vi "Two Way Event Recorder Init VISA Comms.vi"(8 "error in (no error)":errorcluster, 11 "Device Ref in":T1 format="%.0x") -> (0 "error out":errorcluster, 3 "Visa reference out":refnum<visa-resource-name>)   [LabVIEW 2017, in "Two Way Event Recorder Custom Device.lvlib"]
uses:
  Two Way Event Recorder Custom Device.lvlib
  <vilib>/NI Veristand/Custom Device API/Custom Device Item Ref.ctl
  Two Way Event Recorder Property Lookup.vi
  <vilib>/NI Veristand/Custom Device API/Get Item Property (String).vi
  <vilib>/NI Veristand/Custom Device API/Get Item Property (U32).vi
  <vilib>/NI Veristand/Custom Device API/Get Item Property (U16).vi
  <vilib>/NI Veristand/Custom Device API/Custom Device API.lvlib
panel:
  in  "Serial Settings:Wire Mode":i16(ring)=-1 items=["Unknown"=-1, "RS485/Wire4"=0, "RS485/Wire2-EchoDTR"=1, "RS485/Wire2-CtrlDTR"=2, "RS485/Wire2-Auto"=3, "RS232/DTE"=128, "RS232/DCE"=129, "RS232/Auto"=130]
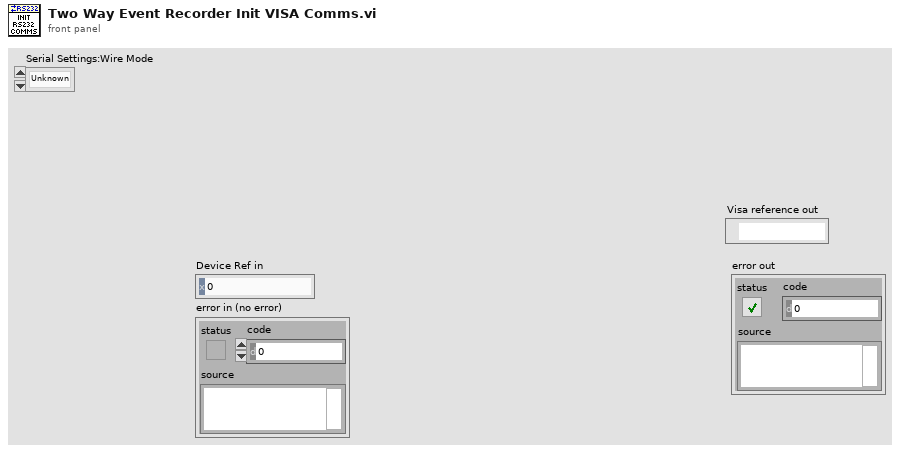
[diagram p1: front panel]
types:
  T1 = typedef "Custom Device API.lvlib/Custom Device Item Ref.ctl" = u64
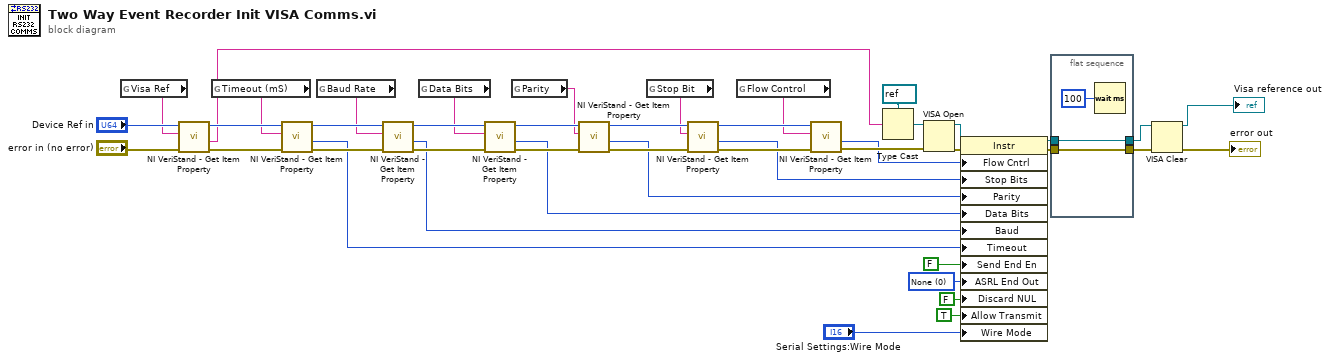
[diagram p0: block diagram]
diagram:
  w4 = u16 0 items=["None", "Last Bit", "TermChar", "Break"] ("Serial Settings:End Mode for Writes")
  n1 = global read "Two Way Event Recorder Property Lookup.vi" "Visa Ref"() -> (w18:string)
  n2 = call-poly <vilib>:"NI VeriStand - Get Item Property.vi"("error in (no error)"="error in (no error)", "Property Name"=w18, "Item Ref in"="Device Ref in") -> ("error out"=w42:errorcluster, "Value"=w31:string, "Item Ref out"=w44:T1)  [unwired: 5 in, 1 out]
  n3 = global read "Two Way Event Recorder Property Lookup.vi" "Timeout (mS)"() -> (w17:string)
  n4 = call-poly <vilib>:"NI VeriStand - Get Item Property.vi"("error in (no error)"=w42, "Property Name"=w17, "Item Ref in"=w44) -> ("error out"=w40:errorcluster, "Value"=w21:u32, "Item Ref out"=w43:T1)  [unwired: 5 in, 1 out]
  n5 = global read "Two Way Event Recorder Property Lookup.vi" "Baud Rate"() -> (w16:string)
  n6 = call-poly <vilib>:"NI VeriStand - Get Item Property.vi"("error in (no error)"=w40, "Property Name"=w16, "Item Ref in"=w43) -> ("error out"=w39:errorcluster, "Value"=w22:u32, "Item Ref out"=w41:T1)  [unwired: 5 in, 1 out]
  n7 = global read "Two Way Event Recorder Property Lookup.vi" "Data Bits"() -> (w15:string)
  n8 = call-poly <vilib>:"NI VeriStand - Get Item Property.vi"("error in (no error)"=w39, "Property Name"=w15, "Item Ref in"=w41) -> ("error out"=w38:errorcluster, "Value"=w23:u16, "Item Ref out"=w37:T1)  [unwired: 5 in, 1 out]
  n9 = global read "Two Way Event Recorder Property Lookup.vi" "Parity"() -> (w14:string)
  n10 = call-poly <vilib>:"NI VeriStand - Get Item Property.vi"("error in (no error)"=w38, "Property Name"=w14, "Item Ref in"=w37) -> ("error out"=w35:errorcluster, "Value"=w24:u16, "Item Ref out"=w36:T1)  [unwired: 5 in, 1 out]
  n11 = global read "Two Way Event Recorder Property Lookup.vi" "Stop Bit"() -> (w13:string)
  n12 = call-poly <vilib>:"NI VeriStand - Get Item Property.vi"("error in (no error)"=w35, "Property Name"=w13, "Item Ref in"=w36) -> ("error out"=w34:errorcluster, "Value"=w25:u16, "Item Ref out"=w33:T1)  [unwired: 5 in, 1 out]
  n13 = global read "Two Way Event Recorder Property Lookup.vi" "Flow Control"() -> (w12:string)
  n14 = call-poly <vilib>:"NI VeriStand - Get Item Property.vi"("error in (no error)"=w34, "Property Name"=w12, "Item Ref in"=w33) -> ("error out"=w28:errorcluster, "Value"=w26:u16)  [unwired: 5 in, 2 out]
  n15 = Type Cast(type=refnum<visa-resource-name> refnum ("reference"), x=w31) -> (*(type *) &x=w30:refnum<visa-resource-name>)
  n16 = VISA Open(error in (no error)=w28, VISA resource name=w30) -> (VISA resource name=w27:refnum<visa-resource-name>, error out=w29:errorcluster)  [unwired: 3 in]
  n17 = property class="Instr"(reference=w27, error in=w29, "Flow Cntrl"=w26, "Stop Bits"=w25, "Parity"=w24, "Data Bits"=w23, "Baud"=w22, "Timeout"=w21, "Send End En"=FALSE ("Message Based Settings:Send End Enable"), "ASRL End Out"=w4, "Discard NUL"=FALSE ("Serial Settings:Discard NUL Characters"), "Allow Transmit"=TRUE ("Serial Settings:Allow Transmit"), "Wire Mode"="Serial Settings:Wire Mode") -> (reference out=w10:refnum<visa-resource-name>, error out=w11:errorcluster)
  n18 = flat-sequence {
    tunnel: w11 -> [w46]
    tunnel: w10 -> [w47]
    tunnel: [w47] -> w8
    tunnel: [w46] -> w9
    frame #0 {
      n19 = Wait (ms)(milliseconds to wait=u32 100) -> ()  [unwired: 1 out]
    }
  }
  n20 = VISA Clear(VISA resource name=w8, error in (no error)=w9) -> (VISA resource name out=→"Visa reference out":refnum<visa-resource-name>, error out=→"error out":errorcluster)
